vi "String Reversal.vi"() -> ()   [LabVIEW 2026]
panel:
  out "Reversed String":string
  in  "Input String":string
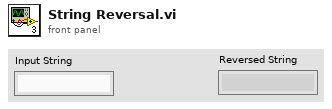
[diagram p1: front panel]
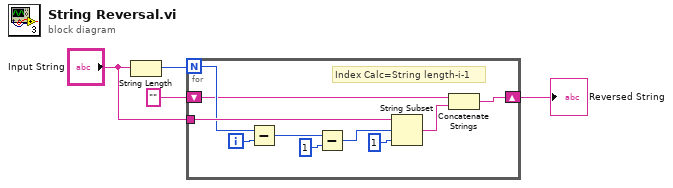
[diagram p0: block diagram]
diagram:
  n1 = String Length(string="Input String") -> (length=w4:i32)
  n2 = for {
    N: w4 -> [w9]
    tunnel: "Input String" -> [w11]
    shift-right: [w5] -> w1
    shift-left: "" -> [w7]
    i -> [w14]
    # "Index Calc=String length-i-1"
    n3 = Subtract(x=w9, y=w14) -> (x-y=w13:i32)
    n4 = Subtract(x=w13, y=1) -> (x-y=w10:i32)
    n5 = String Subset(string=w11, offset (0)=w10, length (rest)=1 ("length (rest)")) -> (substring=w6:string)
    n6 = Concatenate Strings(w7, w6) -> (w5:string)
  }
  "Reversed String" <- w1
